vi "TurnTable Control Method.vi"(8 "error in (no error)":errorcluster caption="에러 입력(에러 없음)", 10 "Turn Table Info":T1, 11 "Instrument Manager 입력":refnum<class "Instrument Manager.lvclass">) -> (0 "error out":errorcluster caption="에러 출력", 3 "Instrument Manager 출력":refnum<class "Instrument Manager.lvclass">)   [LabVIEW 2023, in "Instrument Manager.lvclass"]
uses:
  Instrument Manager.lvclass
  Instrument Manager.lvclass/Instrument Manager.ctl
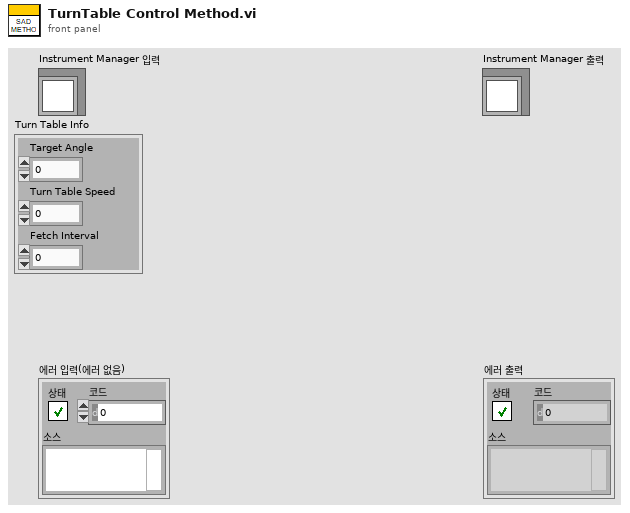
[diagram p1: front panel]
types:
  T1 = cluster{"Target Angle":dbl, "Turn Table Speed":i32, "Fetch Interval":i32}
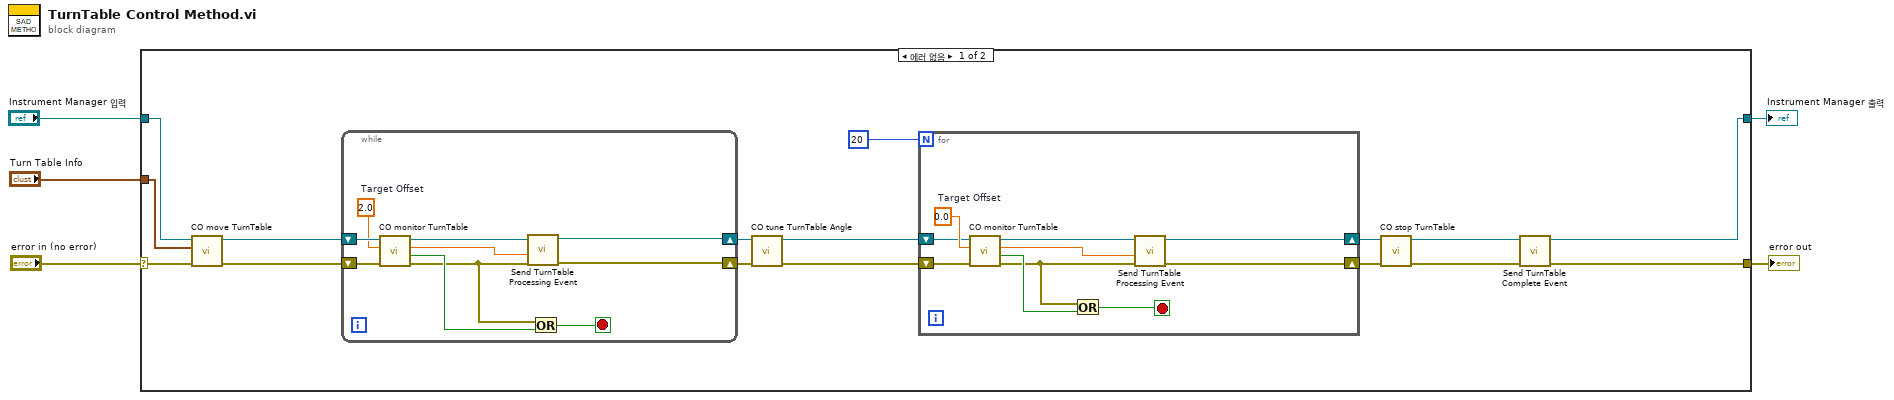
[diagram p0: block diagram]
diagram:
  n1 = case shown="에러 없음" "error in (no error)" {
    selector: "error in (no error)" -> [w9 w43]
    tunnel: [w12 w43] -> w4
    tunnel: [w11 w42] -> w2
    tunnel: "Instrument Manager 입력" -> [w8 w42]
    tunnel: "Turn Table Info" -> [w6 _]
    frame No Error {
      n2 = call "CO move TurnTable.vi"("error in (no error)"=w9, "Turn Table Info"=w6, "Instrument Manager 입력"=w8) -> ("error out"=w10:errorcluster, "Instrument Manager 출력"=w7:refnum<class "Instrument Manager.lvclass">)  [unwired: 7 in]
      n3 = while {
        shift-right: [w33] -> w15
        shift-left: w10 -> [w39]
        shift-right: [w32] -> w14
        shift-left: w7 -> [w40]
        stop <- w41 stop-if-true
        w37 = 2.0  # Target Offset
        n4 = call "CO monitor TurnTable.vi"("error in (no error)"=w39, "Target Offset"=w37, "Instrument Manager 입력"=w40) -> ("error out"=w34:errorcluster, "In Offset Range?"=w38:bool, "Current Angle"=w35:dbl, "Instrument Manager 출력"=w36:refnum<class "Instrument Manager.lvclass">)  [unwired: 4 in]
        n5 = call "Send TurnTable Processing Event.vi"("error in (no error)"=w34, "숫자형"=w35, "Instrument Manager 입력"=w36) -> ("error out"=w33:errorcluster, "Instrument Manager 출력"=w32:refnum<class "Instrument Manager.lvclass">)  [unwired: 7 in]
        n6 = Or(x=w34, y=w38) -> (x .or. y?=w41:bool)
      }
      n7 = call "CO tune TurnTable Angle.vi"("error in (no error)"=w15, "Instrument Manager 입력"=w14) -> ("error out"=w17:errorcluster, "Instrument Manager 출력"=w16:refnum<class "Instrument Manager.lvclass">)  [unwired: 8 in]
      n8 = for {
        N: 20 -> [_]
        shift-right: [w23] -> w19
        shift-left: w17 -> [w30]
        shift-right: [w24] -> w18
        shift-left: w16 -> [w29]
        stop <- w27 stop-if-true
        w31 = 0.0  # Target Offset
        n9 = call "CO monitor TurnTable.vi"("error in (no error)"=w30, "Target Offset"=w31, "Instrument Manager 입력"=w29) -> ("error out"=w26:errorcluster, "In Offset Range?"=w28:bool, "Current Angle"=w22:dbl, "Instrument Manager 출력"=w25:refnum<class "Instrument Manager.lvclass">)  [unwired: 4 in]
        n10 = Or(x=w26, y=w28) -> (x .or. y?=w27:bool)
        n11 = call "Send TurnTable Processing Event.vi"("error in (no error)"=w26, "숫자형"=w22, "Instrument Manager 입력"=w25) -> ("error out"=w23:errorcluster, "Instrument Manager 출력"=w24:refnum<class "Instrument Manager.lvclass">)  [unwired: 7 in]
      }
      n12 = call "CO stop TurnTable.vi"("error in (no error)"=w19, "Instrument Manager 입력"=w18) -> ("error out"=w21:errorcluster, "Instrument Manager 출력"=w20:refnum<class "Instrument Manager.lvclass">)  [unwired: 8 in]
      n13 = call "Send TurnTable Complete Event.vi"("error in (no error)"=w21, "Instrument Manager 입력"=w20) -> ("error out"=w12:errorcluster, "Instrument Manager 출력"=w11:refnum<class "Instrument Manager.lvclass">)  [unwired: 8 in]
    }
    frame Error {
    }
  }
  "error out" <- w4
  "Instrument Manager 출력" <- w2
